vi "Redim.vi"(8 "error in":errorcluster, 9 "Columns":i32=1, 10 "Rows":i32=2, 11 "Sourcegrid in":refnum<class "SourceGrid.lvclass">) -> (0 "error out":errorcluster, 3 "Sourcegrid out":refnum<class "SourceGrid.lvclass">)   [LabVIEW 2020, in "SourceGrid.lvlib" / "SourceGrid.lvclass"]
doc: "Set the number of columns and rows"
uses:
  SourceGrid.lvclass
  SourceGrid.lvclass/SourceGrid.ctl
  D:/git/Sourcegrid-LabVIEW/source/SourceGrid.dll
  SourceGrid.dll
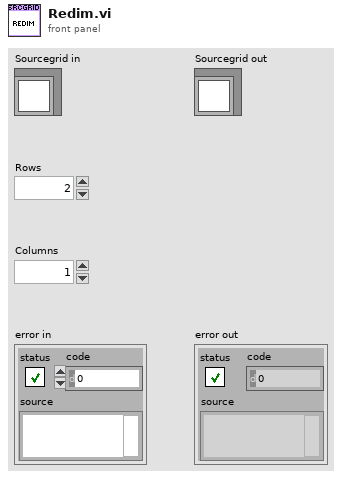
[diagram p1: front panel]
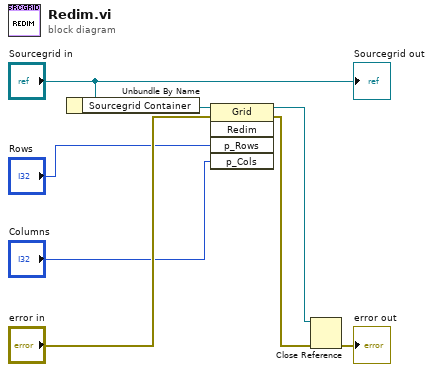
[diagram p0: block diagram]
diagram:
  n1 = Unbundle By Name("Sourcegrid in") -> ("Sourcegrid Container"=w7:refnum<k24>)
  n2 = invoke class="Grid" method="Redim"(reference=w7, error in="error in", "p_Rows"="Rows", "p_Cols"="Columns") -> (reference out=w1:refnum<k24>, error out=w5:errorcluster)  [unwired: 1 in, 3 out]
  n3 = Close Reference(reference=w1, error in (no error)=w5) -> (error out=→"error out":errorcluster)
  "Sourcegrid out" <- "Sourcegrid in"
